vi "H11_TDMS_vs_CSV.vi"() -> ()   [LabVIEW 2026]
doc: "Use this template to build a VI to use as a subVI."
panel:
  out "T3 first value":dbl
  out "T3 samples read":i32
  out "error out":errorcluster
  in  "csv file":path
  in  "tdms file":path
  in  "samples per channel":i32
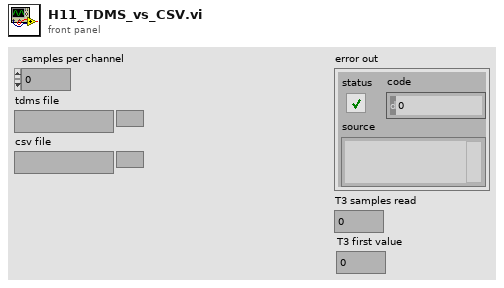
[diagram p1: front panel]
types:
  T1 = enum16{"open", "open or create", "create or replace", "create", "open (read-only)"}
  T2 = enum16{"open", "replace", "create", "open or create", "replace or create", "replace or create with confirmation"}
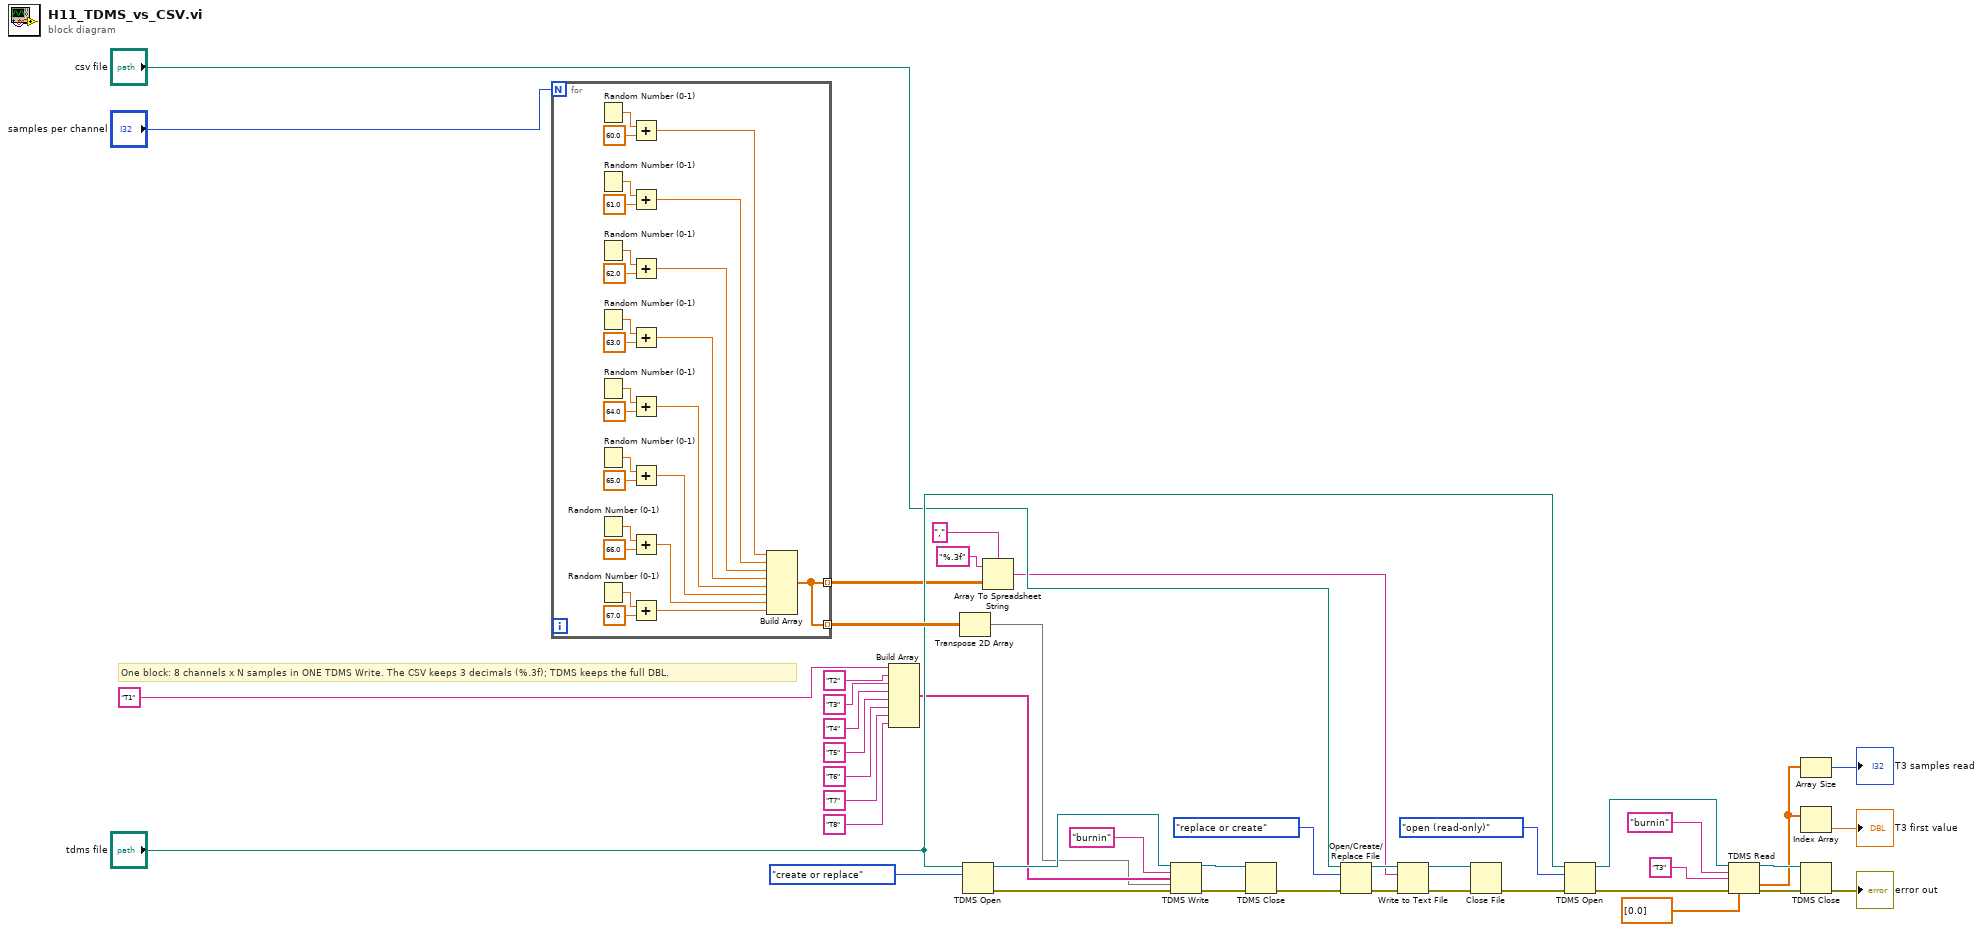
[diagram p0: block diagram]
diagram:
  # "One block: 8 channels x N samples in ONE TDMS Write. The CSV keeps 3 decimals (%.3f); TDMS keeps the full DBL."
  n1 = for {
    N: "samples per channel" -> [_]
    tunnel: [w44] -> w42 mode=indexing
    tunnel: [w44] -> w22 mode=indexing
    n2 = Random Number (0-1)() -> (number: 0 to 1=w68:dbl)
    n3 = Random Number (0-1)() -> (number: 0 to 1=w66:dbl)
    n4 = Random Number (0-1)() -> (number: 0 to 1=w64:dbl)
    n5 = Random Number (0-1)() -> (number: 0 to 1=w62:dbl)
    n6 = Random Number (0-1)() -> (number: 0 to 1=w60:dbl)
    n7 = Random Number (0-1)() -> (number: 0 to 1=w58:dbl)
    n8 = Random Number (0-1)() -> (number: 0 to 1=w56:dbl)
    n9 = Random Number (0-1)() -> (number: 0 to 1=w54:dbl)
    n10 = Add(x=w68, y=60.0) -> (x+y=w52:dbl)
    n11 = Add(x=w66, y=61.0) -> (x+y=w51:dbl)
    n12 = Add(x=w64, y=62.0) -> (x+y=w50:dbl)
    n13 = Add(x=w62, y=63.0) -> (x+y=w49:dbl)
    n14 = Add(x=w60, y=64.0) -> (x+y=w48:dbl)
    n15 = Add(x=w58, y=65.0) -> (x+y=w47:dbl)
    n16 = Add(x=w56, y=66.0) -> (x+y=w46:dbl)
    n17 = Add(x=w54, y=67.0) -> (x+y=w45:dbl)
    n18 = Build Array(w52, w51, w50, w49, w48, w47, w46, w45) -> (w44:dbl[])
  }
  n19 = Build Array("T1", "T2", "T3", "T4", "T5", "T6", "T7", "T8") -> (w28:string[])
  n20 = Transpose 2D Array(2D array=w42) -> (transposed array=w27:dbl[][])
  n21 = TDMS Open(10:T1."create or replace" ("operation (0:open)"), 11:"tdms file") -> (0:w30:errorcluster, 3:w31:refnum<k34>)  [unwired: 5 in]
  n22 = Array To Spreadsheet String(delimiter (Tab)=",", array=w22, 3:"%.3f") -> (spreadsheet string=w16:string)
  n23 = TDMS Write(0:w31, 5:"burnin", 7:w28, 9:w27, 11:w30) -> (4:w26:refnum<k34>, 15:w25:errorcluster)  [unwired: 1 in, 2 out]
  n24 = TDMS Close(8:w25, 11:w26) -> (0:w19:errorcluster)  [unwired: 1 out]
  n25 = Open/Create/Replace File(file path (use dialog)="csv file", error in=w19, operation (0:open)=T2."replace or create") -> (refnum out=w18:refnum<file>, error out=w17:errorcluster)  [unwired: 3 in, 1 out]
  n26 = Write to Text File(file (use dialog)=w18, text=w16, error in=w17) -> (refnum out=w15:refnum<file>, error out=w14:errorcluster)  [unwired: 1 in, 1 out]
  n27 = Close File(refnum=w15, error in=w14) -> (error out=w12:errorcluster)  [unwired: 1 out]
  n28 = TDMS Open(8:w12, 10:T1."open (read-only)" ("operation (0:open)"), 11:"tdms file") -> (0:w10:errorcluster, 3:w11:refnum<k34>)  [unwired: 4 in]
  n29 = TDMS Read(0:w11, 5:"burnin", 7:"T3", 11:w10, 12:dbl[] [0.0] ("Y")) -> (4:w6:refnum<k34>, 10:w3:dbl[], 15:w5:errorcluster)  [unwired: 3 in, 3 out]
  n30 = Array Size(array=w3) -> (size(s)=→"T3 samples read":i32)
  n31 = Index Array(array=w3) -> (element=→"T3 first value":dbl)  [unwired: 1 in]
  n32 = TDMS Close(8:w5, 11:w6) -> (0:→"error out":errorcluster)  [unwired: 1 out]
